vi "250-2.vi"() -> ()   [LabVIEW 2025]
uses:
  <vilib>/Platform/TimedLoop/XDataNode/timing_clust.ctl
  <vilib>/Platform/TimedLoop/XDataNode/nitl_modes.ctl
  <vilib>/Platform/TimedLoop/XDataNode/wakeup.ctl
  <vilib>/eio/utilities/niEioResolveVilibRelativePath.vi
  <vilib>/rvi/interface/RandomDataEmulation/niFpgaRandomDataHandleErrors.vi
  <vilib>/rvi/Memory/Memory_Emulation/nirvimemoryFastEmulation.vi
  <vilib>/rvi/Memory/Memory_Emulation/nirvimemoryEmulation.vi
  <vilib>/rvi/Emulation/niFpgaEmulationIsFPGAContextNoSignature.vi
  <vilib>/rvi/DataTransferAndStorage/Container/Common/niFpgaContainerGetUniqueNameForEmu.vi
  <vilib>/rvi/Emulation/niFpgaProcessEmulError.vi
  <vilib>/rvi/Emulation/niFpgaSctlEmulationGetInTimedLoop.vi
  <vilib>/rvi/errors/nirviReportUnexpectedCaseInternalError (U32).vi
  <vilib>/rvi/Emulation/niFpgaEmulationReportErrorSimple.vi
  <vilib>/rvi/Emulation/niFpgaGetClockAttributes.vi
  <vilib>/rvi/Emulation/niFpgaCriticalErrorInLSC.vi
  <vilib>/rvi/linearAlgebra/MatrixMultiply/simVIs/SubVI/nifxpla_MatrixMultiply_SimMatrixSizes.vi
  <vilib>/rvi/linearAlgebra/MatrixMultiply/simVIs/SubVI/nifxpla_MatrixMultiply_Sim4WireAdapterVector.vi
  <vilib>/rvi/linearAlgebra/MatrixMultiply/simVIs/SubVI/nifxpla_MatrixMultiply_SimFrameHandShake.vi
  <vilib>/rvi/linearAlgebra/MatrixMultiply/simVIs/SubVI/nifxpla_MatrixMultiply_SimEndlessCounter.vi
  <vilib>/rvi/linearAlgebra/MatrixMultiply/simVIs/SubVI/nifxpla_MatrixMultiply_SimVectorDataBuffer.vi
  <vilib>/rvi/ClientSDK/Core/DevComputerLib/Private/Multiply(dfxp64).vi
  <vilib>/rvi/ClientSDK/Core/DevComputerLib/Private/Dfxp128ToDfxp256.vi
  <vilib>/rvi/ClientSDK/Core/DevComputerLib/Private/Add(dfxp256).vi
  <vilib>/rvi/ClientSDK/Core/DevComputerLib/Private/Subtract(dfxp256).vi
  <vilib>/rvi/ClientSDK/Core/DevComputerLib/Private/ToDfxp64(dfxp256).vi
  <vilib>/rvi/DataTransferAndStorage/Container/XNode/niFpgaContainer.xnode
  <vilib>/rvi/interface/RandomDataEmulation/nirviRandomDataFpgaReadWriteTemplate.vi
  <vilib>/platform/TimedLoop/XDataNode/XDataNode.xnode
  <vilib>/rvi/linearAlgebra/MatrixMultiply/XNode/nifxpla_MatrixMultiply.xnode
  <vilib>/rvi/linearAlgebra/MatrixMultiply/simVIs/nifxpla_MatrixMultiply_SimTemplateEinEout.vi
  <vilib>/rvi/linearAlgebra/MatrixMultiply/simVIs/nifxpla_MatrixMultiply_SimTemplateEinVout.vi
  <vilib>/rvi/linearAlgebra/MatrixMultiply/simVIs/nifxpla_MatrixMultiply_SimTemplateVinEout.vi
  <vilib>/rvi/linearAlgebra/MatrixMultiply/simVIs/nifxpla_MatrixMultiply_SimTemplateVinVout.vi
  <vilib>/Platform/TimedLoop/XDataNode/XDNodeRunTimeDep.lvlib
panel:
  out "Latency":u32
  out "Cycle Count":i32
  out "C1":fxp<+/-,32,16>[](array[numeric])
  out "C1+B":fxp<+/-,33,17>[](array[numeric])
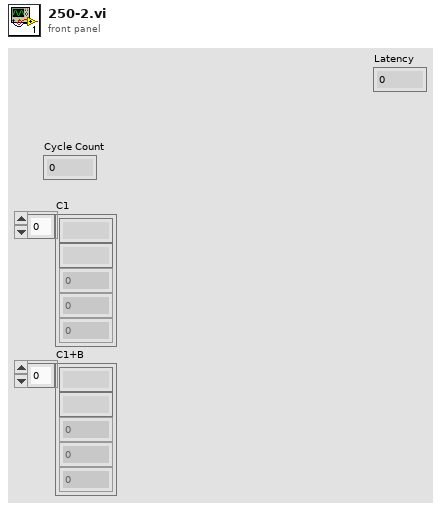
[diagram p1: front panel]
types:
  T1 = typedef "XDNodeRunTimeDep.lvlib/timing_clust.ctl" = cluster{"Expected End [f-1]":u64, "Actual End [f-1]":u64, "Finished Late? [f-1]":bool, "Expected End [i-1]":u64, "Actual End [i-1]":u64, "Finished Late? [i-1]":bool, "Expected Start [i]":u64, "Actual Start [i]":u64, "Expected Start [f]":u64, "Actual Start [f]":u64, "Source Name":string, "Structure Name":string, "Period":i64, "Deadline":i64, "Offset":i64, "Start":i64, "Priority":i32, "Timeout":i32, "Mode":T2, "Wakeup Reason":T3, "Error":errorcluster, "Source Type":string, "Secondary Source Type":string, "Global End Time":u64, "Global Start Time":u64, "Frame Duration":u64, "Iteration Duration":u64, "Assigned CPU":i32, "I/O Scan Engine Mode":u32}
  T2 = typedef "XDNodeRunTimeDep.lvlib/nitl_modes.ctl" = enum32{"No Change", "Process missed periods, maintain original phase", "Discard missed periods, maintain original phase", "Process missed periods, ignore original phase", "Discard missed periods, ignore original phase"}
  T3 = typedef "XDNodeRunTimeDep.lvlib/wakeup.ctl" = enum32{"Normal", "Aborted", "Asynchronous wakeup", "Timing source error", "Timed loop error", "Timeout"}
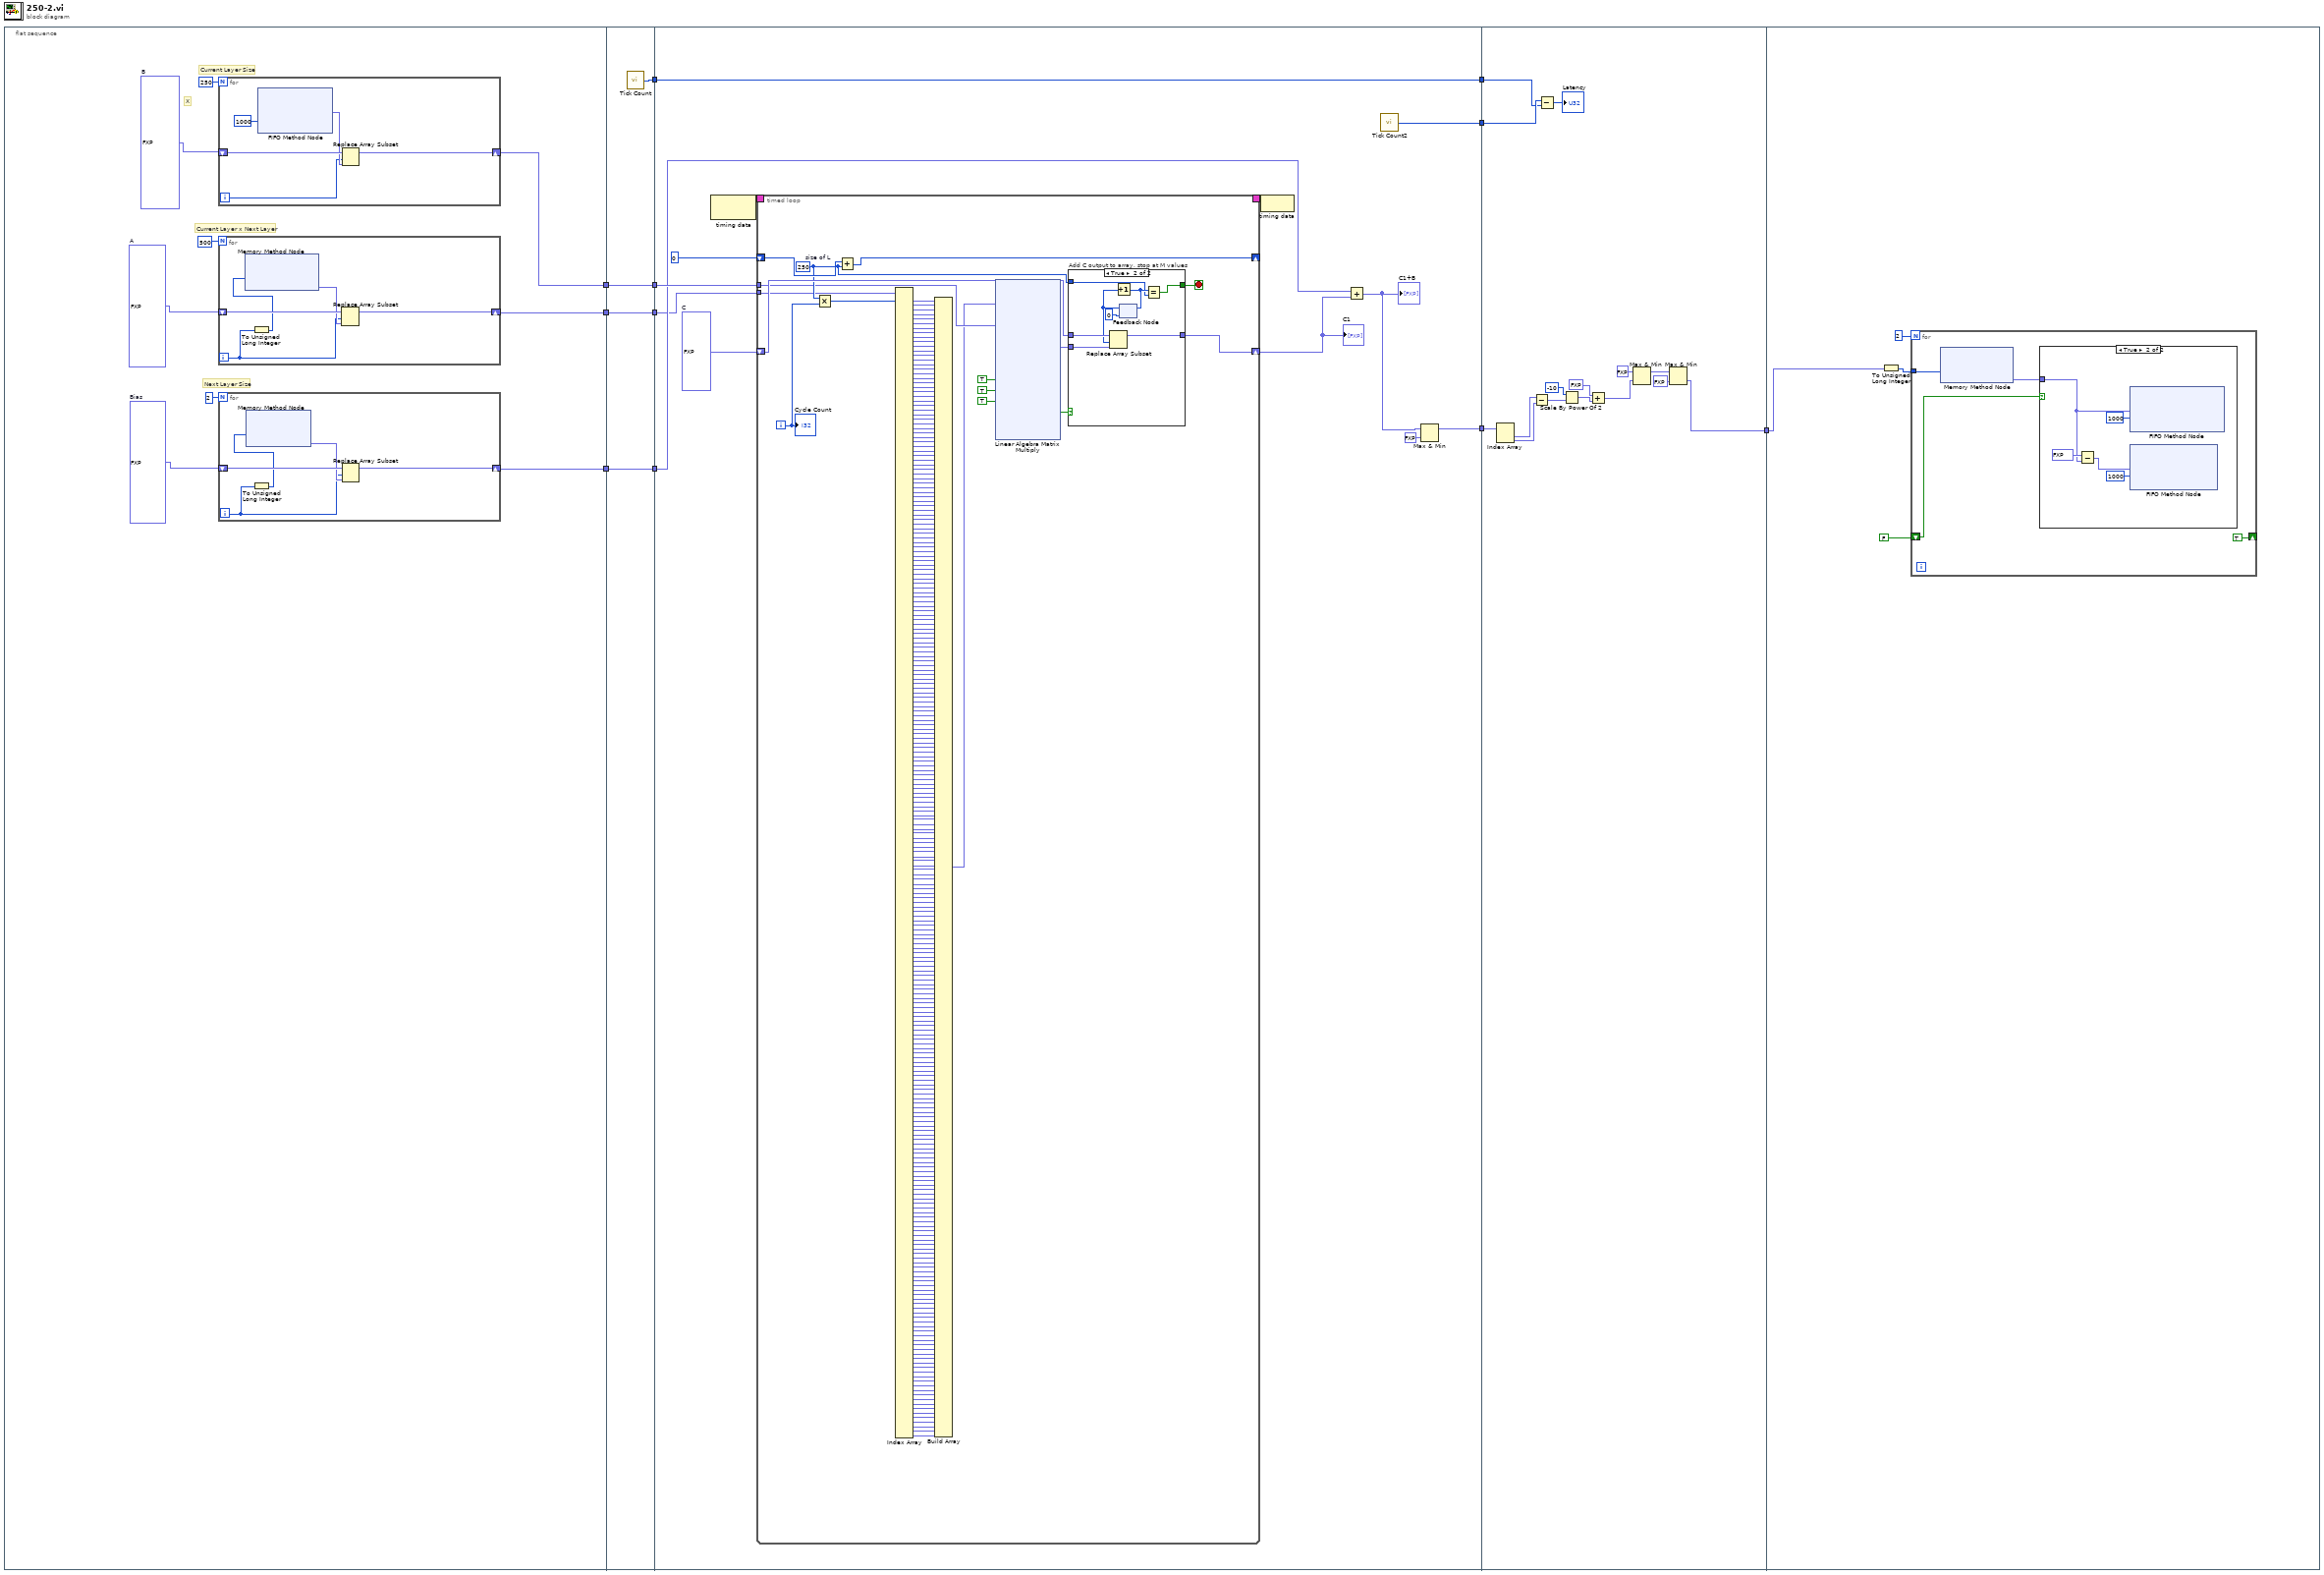
[diagram p0: block diagram]
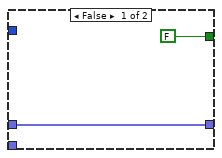
[diagram p2: hidden frame]
diagram:
  n1 = flat-sequence {
    tunnel: [w16] -> w7
    tunnel: [w13] -> w5
    tunnel: [w12] -> w2
    tunnel: [w39] -> w11
    tunnel: [w38] -> w8
    tunnel: w7 -> [w38]
    tunnel: [w37] -> w6
    tunnel: w5 -> [w37]
    tunnel: w2 -> [w36]
    tunnel: [w36] -> w1
    tunnel: [w52] -> w10
    tunnel: [w51] -> w9
    tunnel: [w49] -> w4
    tunnel: w11 -> [w52]
    tunnel: w8 -> [w43]
    tunnel: w6 -> [w42]
    tunnel: w1 -> [w40]
    tunnel: w10 -> [w346]
    tunnel: w9 -> [w347]
    tunnel: w4 -> [w344]
    tunnel: [w333] -> w3
    tunnel: w3 -> [w349]
    frame #0 {
      w14 = fxp<+/-,32,16>[] [0.0, 0.0]  # Bias
      w17 = fxp<+/-,32,16>[] [0.0, 0.0, 0.0, 0.0, 0.0, 0.0, 0.0, 0.0, 0.0, 0.0, 0.0, 0.0, 0.0, 0.0, 0.0, 0.0, 0.0, 0.0, 0.0, 0.0, 0.0, 0.0, 0.0, 0.0, 0.0, 0.0, 0.0, 0.0, 0.0, 0.0, 0.0, 0.0, 0.0, 0.0, 0.0, 0.0, 0.0, 0.0, 0.0, 0.0, 0.0, 0.0, 0.0, 0.0, 0.0, 0.0, 0.0, 0.0, 0.0, 0.0, 0.0, 0.0, 0.0, 0.0, 0.0, 0.0, 0.0, 0.0, 0.0, 0.0, 0.0, 0.0, 0.0, 0.0, 0.0, 0.0, 0.0, 0.0, 0.0, 0.0, 0.0, 0.0, 0.0, 0.0, 0.0, 0.0, 0.0, 0.0, 0.0, 0.0, 0.0, 0.0, 0.0, 0.0, 0.0, 0.0, 0.0, 0.0, 0.0, 0.0, 0.0, 0.0, 0.0, 0.0, 0.0, 0.0, 0.0, 0.0, 0.0, 0.0, 0.0, 0.0, 0.0, 0.0, 0.0, 0.0, 0.0, 0.0, 0.0, 0.0, 0.0, 0.0, 0.0, 0.0, 0.0, 0.0, 0.0, 0.0, 0.0, 0.0, 0.0, 0.0, 0.0, 0.0, 0.0, 0.0, 0.0, 0.0, 0.0, 0.0, 0.0, 0.0, 0.0, 0.0, 0.0, 0.0, 0.0, 0.0, 0.0, 0.0, 0.0, 0.0, 0.0, 0.0, 0.0, 0.0, 0.0, 0.0, 0.0, 0.0, 0.0, 0.0, 0.0, 0.0, 0.0, 0.0, 0.0, 0.0, 0.0, 0.0, 0.0, 0.0, 0.0, 0.0, 0.0, 0.0, 0.0, 0.0, 0.0, 0.0, 0.0, 0.0, 0.0, 0.0, 0.0, 0.0, 0.0, 0.0, 0.0, 0.0, 0.0, 0.0, 0.0, 0.0, 0.0, 0.0, 0.0, 0.0, 0.0, 0.0, 0.0, 0.0, 0.0, 0.0, 0.0, 0.0, 0.0, 0.0, 0.0, 0.0, 0.0, 0.0, 0.0, 0.0, 0.0, 0.0, 0.0, 0.0, 0.0, 0.0, 0.0, 0.0, 0.0, 0.0, 0.0, 0.0, 0.0, 0.0, 0.0, 0.0, 0.0, 0.0, 0.0, 0.0, 0.0, 0.0, 0.0, 0.0, 0.0, 0.0, 0.0, 0.0, 0.0, 0.0, 0.0, 0.0, 0.0, 0.0, 0.0, 0.0, 0.0, 0.0, 0.0, 0.0, 0.0, 0.0, 0.0, 0.0, 0.0, 0.0, 0.0, 0.0, 0.0, 0.0, 0.0, 0.0, 0.0, 0.0, 0.0, 0.0, 0.0, 0.0, 0.0, 0.0, 0.0, 0.0, 0.0, 0.0, 0.0, 0.0, 0.0, 0.0, 0.0, 0.0, 0.0, 0.0, 0.0, 0.0, 0.0, 0.0, 0.0, 0.0, 0.0, 0.0, 0.0, 0.0, 0.0, 0.0, 0.0, 0.0, 0.0, 0.0, 0.0, 0.0, 0.0, 0.0, 0.0, 0.0, 0.0, 0.0, 0.0, 0.0, 0.0, 0.0, 0.0, 0.0, 0.0, 0.0, 0.0, 0.0, 0.0, 0.0, 0.0, 0.0, 0.0, 0.0, 0.0, 0.0, 0.0, 0.0, 0.0, 0.0, 0.0, 0.0, 0.0, 0.0, 0.0, 0.0, 0.0, 0.0, 0.0, 0.0, 0.0, 0.0, 0.0, 0.0, 0.0, 0.0, 0.0, 0.0, 0.0, 0.0, 0.0, 0.0, 0.0, 0.0, 0.0, 0.0, 0.0, 0.0, 0.0, 0.0, 0.0, 0.0, 0.0, 0.0, 0.0, 0.0, 0.0, 0.0, 0.0, 0.0, 0.0, 0.0, 0.0, 0.0, 0.0, 0.0, 0.0, 0.0, 0.0, 0.0, 0.0, 0.0, 0.0, 0.0, 0.0, 0.0, 0.0, 0.0, 0.0, 0.0, 0.0, 0.0, 0.0, 0.0, 0.0, 0.0, 0.0, 0.0, 0.0, 0.0, 0.0, 0.0, 0.0, 0.0, 0.0, 0.0, 0.0, 0.0, 0.0, 0.0, 0.0, 0.0, 0.0, 0.0, 0.0, 0.0, 0.0, 0.0, 0.0, 0.0, 0.0, 0.0, 0.0, 0.0, 0.0, 0.0, 0.0, 0.0, 0.0, 0.0, 0.0, 0.0, 0.0, 0.0, 0.0, 0.0, 0.0, 0.0, 0.0, 0.0, 0.0, 0.0, 0.0, 0.0, 0.0, 0.0, 0.0, 0.0, 0.0, 0.0, 0.0, 0.0, 0.0, 0.0, 0.0, 0.0, 0.0, 0.0, 0.0, 0.0, 0.0, 0.0, 0.0, 0.0, 0.0, 0.0, 0.0, 0.0, 0.0, 0.0, 0.0, 0.0, 0.0, 0.0, 0.0, 0.0, 0.0, 0.0, 0.0, 0.0, 0.0, 0.0, 0.0, 0.0, 0.0, 0.0, 0.0, 0.0, 0.0, 0.0, 0.0, 0.0, 0.0, 0.0, 0.0, 0.0, 0.0, 0.0, 0.0, 0.0, 0.0, 0.0, 0.0, 0.0, 0.0, 0.0, 0.0, 0.0]  # A
      w19 = fxp<+/-,32,16>[] [0.0, 0.0, 0.0, 0.0, 0.0, 0.0, 0.0, 0.0, 0.0, 0.0, 0.0, 0.0, 0.0, 0.0, 0.0, 0.0, 0.0, 0.0, 0.0, 0.0, 0.0, 0.0, 0.0, 0.0, 0.0, 0.0, 0.0, 0.0, 0.0, 0.0, 0.0, 0.0, 0.0, 0.0, 0.0, 0.0, 0.0, 0.0, 0.0, 0.0, 0.0, 0.0, 0.0, 0.0, 0.0, 0.0, 0.0, 0.0, 0.0, 0.0, 0.0, 0.0, 0.0, 0.0, 0.0, 0.0, 0.0, 0.0, 0.0, 0.0, 0.0, 0.0, 0.0, 0.0, 0.0, 0.0, 0.0, 0.0, 0.0, 0.0, 0.0, 0.0, 0.0, 0.0, 0.0, 0.0, 0.0, 0.0, 0.0, 0.0, 0.0, 0.0, 0.0, 0.0, 0.0, 0.0, 0.0, 0.0, 0.0, 0.0, 0.0, 0.0, 0.0, 0.0, 0.0, 0.0, 0.0, 0.0, 0.0, 0.0, 0.0, 0.0, 0.0, 0.0, 0.0, 0.0, 0.0, 0.0, 0.0, 0.0, 0.0, 0.0, 0.0, 0.0, 0.0, 0.0, 0.0, 0.0, 0.0, 0.0, 0.0, 0.0, 0.0, 0.0, 0.0, 0.0, 0.0, 0.0, 0.0, 0.0, 0.0, 0.0, 0.0, 0.0, 0.0, 0.0, 0.0, 0.0, 0.0, 0.0, 0.0, 0.0, 0.0, 0.0, 0.0, 0.0, 0.0, 0.0, 0.0, 0.0, 0.0, 0.0, 0.0, 0.0, 0.0, 0.0, 0.0, 0.0, 0.0, 0.0, 0.0, 0.0, 0.0, 0.0, 0.0, 0.0, 0.0, 0.0, 0.0, 0.0, 0.0, 0.0, 0.0, 0.0, 0.0, 0.0, 0.0, 0.0, 0.0, 0.0, 0.0, 0.0, 0.0, 0.0, 0.0, 0.0, 0.0, 0.0, 0.0, 0.0, 0.0, 0.0, 0.0, 0.0, 0.0, 0.0, 0.0, 0.0, 0.0, 0.0, 0.0, 0.0, 0.0, 0.0, 0.0, 0.0, 0.0, 0.0, 0.0, 0.0, 0.0, 0.0, 0.0, 0.0, 0.0, 0.0, 0.0, 0.0, 0.0, 0.0, 0.0, 0.0, 0.0, 0.0, 0.0, 0.0, 0.0, 0.0, 0.0, 0.0, 0.0, 0.0, 0.0, 0.0, 0.0, 0.0, 0.0, 0.0, 0.0, 0.0, 0.0, 0.0, 0.0, 0.0, 0.0, 0.0, 0.0, 0.0, 0.0, 0.0]  # B
      # "Next Layer Size"
      # "Current Layer Size"
      # "Current Layer x Next Layer"
      # "X"
      n2 = for {
        N: 500 -> [_]
        shift-right: [w29] -> w12
        shift-left: w17 -> [w30]
        i -> [w27]
        n3 = To Unsigned Long Integer(number=w27) -> (unsigned 32bit integer=w26:u32)
        n4 = xnode ("Memory Method Node")("Address"=w26) -> ("Data"=w28:fxp<+/-,32,16>)  [unwired: 1 in, 1 out]
        n5 = Replace Array Subset(array=w30, new element=w28, index=w27) -> (w29:fxp<+/-,32,16>[])
      }
      n6 = for {
        N: 250 -> [_]
        shift-right: [w32] -> w16
        shift-left: w19 -> [w34]
        i -> [w31]
        n7 = xnode ("FIFO Method Node")("Timeout"=1000) -> ("Element"=w33:fxp<+/-,32,16>)  [unwired: 1 in, 2 out]
        n8 = Replace Array Subset(array=w34, new element=w33, index=w31) -> (w32:fxp<+/-,32,16>[])
      }
      n9 = for {
        N: 2 -> [_]
        shift-right: [w24] -> w13
        shift-left: w14 -> [w25]
        i -> [w22]
        n10 = To Unsigned Long Integer(number=w22) -> (unsigned 32bit integer=w21:u32)
        n11 = xnode ("Memory Method Node")("Address"=w21) -> ("Data"=w23:fxp<+/-,32,16>)  [unwired: 1 in, 1 out]
        n12 = Replace Array Subset(array=w25, new element=w23, index=w22) -> (w24:fxp<+/-,32,16>[])
      }
    }
    frame #1 {
      n13 = call "Tick Count"() -> ("Tick Count(Ticks)"=w39:u32)
    }
    frame #2 {
      w46 = fxp<+/-,32,16>[] [0.0, 0.0]  # C
      n14 = node-c288() -> (w48:T1)  [unwired: 1 in]
      n15 = timed-loop {
        timing: w48 -> [_]
        timing-out: [_] -> w47
        shift-right: [w317] -> w44
        shift-left: w46 -> [w316]
        shift-right: [w310] -> _
        shift-left: 0 ("length") -> [w311]
        tunnel: w40 -> [w177]
        tunnel: w43 -> [w176]
        i -> [w297]
        stop <- w315 stop-if-true
        w296 = 250  # size of L
        n16 = Multiply(x=w296, y=w297) -> (x*y=w308:i32)
        n17 = Add(x=w311, y=w296) -> (x+y=w310:i32)
        n18 = Index Array(array=w177, index #1=w308) -> (element #1=w307:fxp<+/-,32,16>, element #2=w306:fxp<+/-,32,16>, element #3=w305:fxp<+/-,32,16>, element #4=w304:fxp<+/-,32,16>, element #5=w303:fxp<+/-,32,16>, element #6=w302:fxp<+/-,32,16>, element #7=w301:fxp<+/-,32,16>, element #8=w300:fxp<+/-,32,16>, element #9=w299:fxp<+/-,32,16>, element #10=w298:fxp<+/-,32,16>, element #11=w295:fxp<+/-,32,16>, element #12=w294:fxp<+/-,32,16>, element #13=w293:fxp<+/-,32,16>, element #14=w292:fxp<+/-,32,16>, element #15=w291:fxp<+/-,32,16>, element #16=w290:fxp<+/-,32,16>, element #17=w289:fxp<+/-,32,16>, element #18=w288:fxp<+/-,32,16>, element #19=w287:fxp<+/-,32,16>, element #20=w286:fxp<+/-,32,16>, element #21=w285:fxp<+/-,32,16>, element #22=w284:fxp<+/-,32,16>, element #23=w283:fxp<+/-,32,16>, element #24=w282:fxp<+/-,32,16>, element #25=w281:fxp<+/-,32,16>, element #26=w280:fxp<+/-,32,16>, element #27=w279:fxp<+/-,32,16>, element #28=w278:fxp<+/-,32,16>, element #29=w277:fxp<+/-,32,16>, element #30=w276:fxp<+/-,32,16>, element #31=w275:fxp<+/-,32,16>, element #32=w274:fxp<+/-,32,16>, element #33=w273:fxp<+/-,32,16>, element #34=w271:fxp<+/-,32,16>, element #35=w272:fxp<+/-,32,16>, element #36=w270:fxp<+/-,32,16>, element #37=w269:fxp<+/-,32,16>, element #38=w268:fxp<+/-,32,16>, element #39=w267:fxp<+/-,32,16>, element #40=w266:fxp<+/-,32,16>, element #41=w265:fxp<+/-,32,16>, element #42=w264:fxp<+/-,32,16>, element #43=w263:fxp<+/-,32,16>, element #44=w262:fxp<+/-,32,16>, element #45=w260:fxp<+/-,32,16>, element #46=w261:fxp<+/-,32,16>, element #47=w259:fxp<+/-,32,16>, element #48=w258:fxp<+/-,32,16>, element #49=w257:fxp<+/-,32,16>, element #50=w256:fxp<+/-,32,16>, element #51=w255:fxp<+/-,32,16>, element #52=w254:fxp<+/-,32,16>, element #53=w253:fxp<+/-,32,16>, element #54=w252:fxp<+/-,32,16>, element #55=w251:fxp<+/-,32,16>, element #56=w250:fxp<+/-,32,16>, element #57=w248:fxp<+/-,32,16>, element #58=w249:fxp<+/-,32,16>, element #59=w247:fxp<+/-,32,16>, element #60=w246:fxp<+/-,32,16>, element #61=w245:fxp<+/-,32,16>, element #62=w244:fxp<+/-,32,16>, element #63=w243:fxp<+/-,32,16>, element #64=w242:fxp<+/-,32,16>, element #65=w241:fxp<+/-,32,16>, element #66=w239:fxp<+/-,32,16>, element #67=w240:fxp<+/-,32,16>, element #68=w237:fxp<+/-,32,16>, element #69=w238:fxp<+/-,32,16>, element #70=w235:fxp<+/-,32,16>, element #71=w236:fxp<+/-,32,16>, element #72=w233:fxp<+/-,32,16>, element #73=w234:fxp<+/-,32,16>, element #74=w232:fxp<+/-,32,16>, element #75=w231:fxp<+/-,32,16>, element #76=w230:fxp<+/-,32,16>, element #77=w229:fxp<+/-,32,16>, element #78=w228:fxp<+/-,32,16>, element #79=w227:fxp<+/-,32,16>, element #80=w226:fxp<+/-,32,16>, element #81=w225:fxp<+/-,32,16>, element #82=w224:fxp<+/-,32,16>, element #83=w223:fxp<+/-,32,16>, element #84=w222:fxp<+/-,32,16>, element #85=w220:fxp<+/-,32,16>, element #86=w221:fxp<+/-,32,16>, element #87=w219:fxp<+/-,32,16>, element #88=w217:fxp<+/-,32,16>, element #89=w218:fxp<+/-,32,16>, element #90=w216:fxp<+/-,32,16>, element #91=w215:fxp<+/-,32,16>, element #92=w214:fxp<+/-,32,16>, element #93=w213:fxp<+/-,32,16>, element #94=w212:fxp<+/-,32,16>, element #95=w211:fxp<+/-,32,16>, element #96=w210:fxp<+/-,32,16>, element #97=w209:fxp<+/-,32,16>, element #98=w208:fxp<+/-,32,16>, element #99=w207:fxp<+/-,32,16>, element #100=w206:fxp<+/-,32,16>, element #101=w205:fxp<+/-,32,16>, element #102=w204:fxp<+/-,32,16>, element #103=w203:fxp<+/-,32,16>, element #104=w202:fxp<+/-,32,16>, element #105=w201:fxp<+/-,32,16>, element #106=w200:fxp<+/-,32,16>, element #107=w199:fxp<+/-,32,16>, element #108=w198:fxp<+/-,32,16>, element #109=w197:fxp<+/-,32,16>, element #110=w195:fxp<+/-,32,16>, element #111=w196:fxp<+/-,32,16>, element #112=w193:fxp<+/-,32,16>, element #113=w194:fxp<+/-,32,16>, element #114=w192:fxp<+/-,32,16>, element #115=w190:fxp<+/-,32,16>, element #116=w191:fxp<+/-,32,16>, element #117=w189:fxp<+/-,32,16>, element #118=w188:fxp<+/-,32,16>, element #119=w187:fxp<+/-,32,16>, element #120=w186:fxp<+/-,32,16>, element #121=w185:fxp<+/-,32,16>, element #122=w184:fxp<+/-,32,16>, element #123=w183:fxp<+/-,32,16>, element #124=w182:fxp<+/-,32,16>, element #125=w181:fxp<+/-,32,16>, element #126=w180:fxp<+/-,32,16>, element #127=w179:fxp<+/-,32,16>, element #128=w178:fxp<+/-,32,16>, element #129=w174:fxp<+/-,32,16>, element #130=w173:fxp<+/-,32,16>, element #131=w172:fxp<+/-,32,16>, element #132=w171:fxp<+/-,32,16>, element #133=w170:fxp<+/-,32,16>, element #134=w169:fxp<+/-,32,16>, element #135=w168:fxp<+/-,32,16>, element #136=w166:fxp<+/-,32,16>, element #137=w167:fxp<+/-,32,16>, element #138=w165:fxp<+/-,32,16>, element #139=w164:fxp<+/-,32,16>, element #140=w163:fxp<+/-,32,16>, element #141=w162:fxp<+/-,32,16>, element #142=w161:fxp<+/-,32,16>, element #143=w160:fxp<+/-,32,16>, element #144=w159:fxp<+/-,32,16>, element #145=w158:fxp<+/-,32,16>, element #146=w157:fxp<+/-,32,16>, element #147=w156:fxp<+/-,32,16>, element #148=w155:fxp<+/-,32,16>, element #149=w154:fxp<+/-,32,16>, element #150=w153:fxp<+/-,32,16>, element #151=w152:fxp<+/-,32,16>, element #152=w151:fxp<+/-,32,16>, element #153=w150:fxp<+/-,32,16>, element #154=w149:fxp<+/-,32,16>, element #155=w148:fxp<+/-,32,16>, element #156=w147:fxp<+/-,32,16>, element #157=w146:fxp<+/-,32,16>, element #158=w145:fxp<+/-,32,16>, element #159=w144:fxp<+/-,32,16>, element #160=w143:fxp<+/-,32,16>, element #161=w142:fxp<+/-,32,16>, element #162=w141:fxp<+/-,32,16>, element #163=w140:fxp<+/-,32,16>, element #164=w139:fxp<+/-,32,16>, element #165=w138:fxp<+/-,32,16>, element #166=w137:fxp<+/-,32,16>, element #167=w136:fxp<+/-,32,16>, element #168=w135:fxp<+/-,32,16>, element #169=w134:fxp<+/-,32,16>, element #170=w133:fxp<+/-,32,16>, element #171=w132:fxp<+/-,32,16>, element #172=w131:fxp<+/-,32,16>, element #173=w130:fxp<+/-,32,16>, element #174=w129:fxp<+/-,32,16>, element #175=w128:fxp<+/-,32,16>, element #176=w127:fxp<+/-,32,16>, element #177=w126:fxp<+/-,32,16>, element #178=w125:fxp<+/-,32,16>, element #179=w124:fxp<+/-,32,16>, element #180=w123:fxp<+/-,32,16>, element #181=w122:fxp<+/-,32,16>, element #182=w121:fxp<+/-,32,16>, element #183=w120:fxp<+/-,32,16>, element #184=w119:fxp<+/-,32,16>, element #185=w118:fxp<+/-,32,16>, element #186=w117:fxp<+/-,32,16>, element #187=w116:fxp<+/-,32,16>, element #188=w115:fxp<+/-,32,16>, element #189=w114:fxp<+/-,32,16>, element #190=w113:fxp<+/-,32,16>, element #191=w112:fxp<+/-,32,16>, element #192=w111:fxp<+/-,32,16>, element #193=w110:fxp<+/-,32,16>, element #194=w109:fxp<+/-,32,16>, element #195=w108:fxp<+/-,32,16>, element #196=w107:fxp<+/-,32,16>, element #197=w106:fxp<+/-,32,16>, element #198=w105:fxp<+/-,32,16>, element #199=w104:fxp<+/-,32,16>, element #200=w103:fxp<+/-,32,16>, element #201=w102:fxp<+/-,32,16>, element #202=w101:fxp<+/-,32,16>, element #203=w100:fxp<+/-,32,16>, element #204=w99:fxp<+/-,32,16>, element #205=w98:fxp<+/-,32,16>, element #206=w97:fxp<+/-,32,16>, element #207=w96:fxp<+/-,32,16>, element #208=w95:fxp<+/-,32,16>, element #209=w94:fxp<+/-,32,16>, element #210=w93:fxp<+/-,32,16>, element #211=w92:fxp<+/-,32,16>, element #212=w91:fxp<+/-,32,16>, element #213=w90:fxp<+/-,32,16>, element #214=w89:fxp<+/-,32,16>, element #215=w88:fxp<+/-,32,16>, element #216=w87:fxp<+/-,32,16>, element #217=w86:fxp<+/-,32,16>, element #218=w85:fxp<+/-,32,16>, element #219=w84:fxp<+/-,32,16>, element #220=w83:fxp<+/-,32,16>, element #221=w82:fxp<+/-,32,16>, element #222=w81:fxp<+/-,32,16>, element #223=w80:fxp<+/-,32,16>, element #224=w79:fxp<+/-,32,16>, element #225=w78:fxp<+/-,32,16>, element #226=w77:fxp<+/-,32,16>, element #227=w76:fxp<+/-,32,16>, element #228=w75:fxp<+/-,32,16>, element #229=w74:fxp<+/-,32,16>, element #230=w73:fxp<+/-,32,16>, element #231=w72:fxp<+/-,32,16>, element #232=w71:fxp<+/-,32,16>, element #233=w70:fxp<+/-,32,16>, element #234=w69:fxp<+/-,32,16>, element #235=w68:fxp<+/-,32,16>, element #236=w67:fxp<+/-,32,16>, element #237=w66:fxp<+/-,32,16>, element #238=w65:fxp<+/-,32,16>, element #239=w64:fxp<+/-,32,16>, element #240=w63:fxp<+/-,32,16>, element #241=w62:fxp<+/-,32,16>, element #242=w61:fxp<+/-,32,16>, element #243=w60:fxp<+/-,32,16>, element #244=w59:fxp<+/-,32,16>, element #245=w58:fxp<+/-,32,16>, element #246=w57:fxp<+/-,32,16>, element #247=w56:fxp<+/-,32,16>, element #248=w55:fxp<+/-,32,16>, element #249=w54:fxp<+/-,32,16>, element #250=w53:fxp<+/-,32,16>)  [unwired: 249 in]
        n19 = Build Array(w307, w306, w305, w304, w303, w302, w301, w300, w299, w298, w295, w294, w293, w292, w291, w290, w289, w288, w287, w286, w285, w284, w283, w282, w281, w280, w279, w278, w277, w276, w275, w274, w273, w271, w272, w270, w269, w268, w267, w266, w265, w264, w263, w262, w260, w261, w259, w258, w257, w256, w255, w254, w253, w252, w251, w250, w248, w249, w247, w246, w245, w244, w243, w242, w241, w239, w240, w237, w238, w235, w236, w233, w234, w232, w231, w230, w229, w228, w227, w226, w225, w224, w223, w222, w220, w221, w219, w217, w218, w216, w215, w214, w213, w212, w211, w210, w209, w208, w207, w206, w205, w204, w203, w202, w201, w200, w199, w198, w197, w195, w196, w193, w194, w192, w190, w191, w189, w188, w187, w186, w185, w184, w183, w182, w181, w180, w179, w178, w174, w173, w172, w171, w170, w169, w168, w166, w167, w165, w164, w163, w162, w161, w160, w159, w158, w157, w156, w155, w154, w153, w152, w151, w150, w149, w148, w147, w146, w145, w144, w143, w142, w141, w140, w139, w138, w137, w136, w135, w134, w133, w132, w131, w130, w129, w128, w127, w126, w125, w124, w123, w122, w121, w120, w119, w118, w117, w116, w115, w114, w113, w112, w111, w110, w109, w108, w107, w106, w105, w104, w103, w102, w101, w100, w99, w98, w97, w96, w95, w94, w93, w92, w91, w90, w89, w88, w87, w86, w85, w84, w83, w82, w81, w80, w79, w78, w77, w76, w75, w74, w73, w72, w71, w70, w69, w68, w67, w66, w65, w64, w63, w62, w61, w60, w59, w58, w57, w56, w55, w54, w53) -> (w175:fxp<+/-,32,16>[])
        n20 = xnode ("Linear Algebra Matrix Multiply")("ar"=w175, "br"=w176, "a valid"=TRUE, "b valid"=TRUE, "ready for output (T)"=TRUE) -> ("cr"=w313:fxp<+/-,64,40>[], "output valid"=w309:bool)  [unwired: 2 in, 4 out]
        n21 = case "Add C output to array, stop at M values" shown="True" w309 {
          tunnel: w313 -> [_ w324]
          tunnel: [w320 w327] -> w317
          tunnel: w316 -> [w320 w328]
          tunnel: [FALSE w325] -> w315
          tunnel: w296 -> [_ w321]
          frame False {
          }
          frame True {
            n22 = feedback #1(0 ("x")) -> (w323:i32)
            n23 = Replace Array Subset(array=w328, new element=w324, index=w323) -> (w327:fxp<+/-,32,16>[])
            n24 = Increment(x=w323) -> (x+1=w322:i32)
            n25 = feedback-in #1(w322) -> ()
            n26 = Equal?(x=w322, y=w321) -> (x = y?=w325:bool)
          }
        }
        "Cycle Count" <- w297
      }
      "C1" <- w44
      n27 = node-c288(w47) -> ()
      n28 = Add(x=w42, y=w44) -> (x+y=w41:fxp<+/-,33,17>[])
      "C1+B" <- w41
      n29 = call "Tick Count2"() -> ("Tick Count(Ticks)"=w51:u32)
      n30 = Max & Min(x=w41, y=fxp<+,1,1> 0.0) -> (max(x,y)=w49:fxp<+/-,33,17>[])  [unwired: 1 out]
    }
    frame #3 {
      n31 = Index Array(array=w344) -> (element #1=w335:fxp<+/-,33,17>, element #2=w334:fxp<+/-,33,17>)  [unwired: 2 in]
      n32 = Subtract(x=w335, y=w334) -> (x-y=w340:fxp<+/-,34,18>)
      n33 = Subtract(x=w347, y=w346) -> (x-y=→"Latency":u32)
      n34 = Scale By Power Of 2(n=i16 -10, x=w340) -> (x*2^n=w341:fxp<+/-,34,18>)
      n35 = Add(x=fxp<+,1,9> 256.0, y=w341) -> (x+y=w342:fxp<+/-,35,19>)
      n36 = Max & Min(x=fxp<+,1,1> 0.0, y=w342) -> (max(x,y)=w343:fxp<+/-,35,19>)  [unwired: 1 out]
      n37 = Max & Min(x=w343, y=fxp<+,9,9> 511.0) -> (min(x,y)=w333:fxp<+/-,35,19>)  [unwired: 1 out]
    }
    frame #4 {
      n38 = To Unsigned Long Integer(number=w349) -> (unsigned 32bit integer=w348:u32)
      n39 = for {
        N: 2 -> [_]
        tunnel: w348 -> [w355]
        shift-right: [TRUE] -> _
        shift-left: FALSE -> [w354]
        n40 = xnode ("Memory Method Node")("Address"=w355) -> ("Data"=w352:fxp<+/-,32,16>)  [unwired: 1 in, 1 out]
        n41 = case shown="True" w354 {
          tunnel: w352 -> [_ w356]
          frame False {
          }
          frame True {
            n42 = Subtract(x=fxp<+,1,16> 32768.0, y=w356) -> (x-y=w360:fxp<+,33,17>)
            n43 = xnode ("FIFO Method Node")("Element"=w356, "Timeout"=1000) -> ()  [unwired: 1 in, 2 out]
            n44 = xnode ("FIFO Method Node")("Element"=w360, "Timeout"=1000) -> ()  [unwired: 1 in, 2 out]
          }
        }
      }
    }
  }
